vi "Copy Set Default Value - Multiple Converter.vi"(11 "error in":errorcluster) -> (15 "error out":errorcluster)   [LabVIEW 2021, in "Converter.lvlib"]
uses:
  Converter.lvlib
  Path Functions/Path Functions.lvlib
  Converter Reusables/Converter Reusables.lvlib
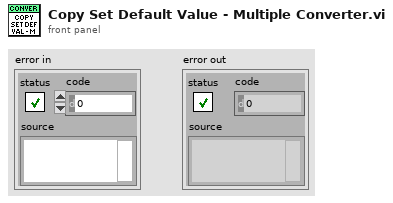
[diagram p1: front panel]
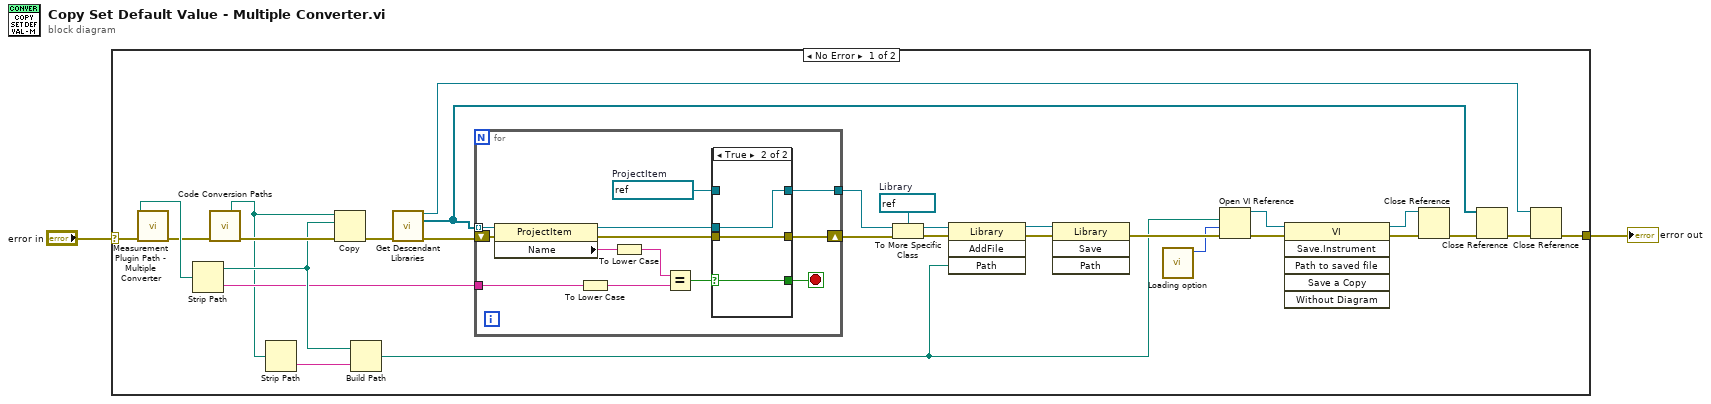
[diagram p0: block diagram]
diagram:
  n1 = case shown="No Error" "error in" {
    selector: "error in" -> [w18 w51]
    tunnel: [w22 w51] -> w2
    frame No Error {
      w12 = refnum<vi> refnum  # Library
      n2 = call "Measurement Plugin Path - Multiple Converter.vi"("error in"=w18) -> ("measurement ui lib"=w19:path, "error out"=w17:errorcluster)  [unwired: 2 in, 11 out]
      n3 = Strip Path(path=w19) -> (stripped path=w29:path, name=w28:string)
      n4 = call "Code Conversion Paths.vi"("error in"=w17) -> ("deafult value setter vi"=w21:path, "error out"=w31:errorcluster)  [unwired: 6 in, 7 out]
      n5 = Strip Path(path=w21) -> (name=w20:string)  [unwired: 1 out]
      n6 = Copy(8:w31, 10:w29, 11:w21) -> (0:w16:errorcluster)  [unwired: 2 in, 2 out]
      n7 = Build Path(base path=w29, name or relative path=w20) -> (appended path=w8:path)
      n8 = call "Get Descendant Libraries.vi"("error in"=w16) -> ("project out"=w23:refnum<vi>, "all descendents"=w27:refnum<vi>[], "error out"=w30:errorcluster)  [unwired: 12 in]
      n9 = for {
        tunnel: w27 -> [w44] mode=indexing
        tunnel: [w37] -> w25
        tunnel: w28 -> [w36]
        shift-right: [w32] -> w10
        shift-left: w30 -> [w35]
        stop <- w38 stop-if-true
        w41 = refnum<vi> refnum  # ProjectItem
        n10 = property class="ProjectItem"(reference=w44, error in=w35) -> (reference out=w40:refnum<vi>, error out=w39:errorcluster, "Name"=w43:string)
        n11 = To Lower Case(string=w36) -> (all lower case string=w33:string)
        n12 = To Lower Case(string=w43) -> (all lower case string=w34:string)
        n13 = Equal?(x=w34, y=w33) -> (x = y?=w42:bool)
        n14 = case shown="True" w42 {
          selector: w42 -> [w46 w49]
          tunnel: w40 -> [_ w50]
          tunnel: [w45 w48] -> w32
          tunnel: [w47 w50] -> w37
          tunnel: w41 -> [w47 _]
          tunnel: [w46 w49] -> w38
          tunnel: w39 -> [w45 w48]
          frame False {
          }
          frame True {
          }
        }
      }
      n15 = To More Specific Class(target class=w12, reference=w25, error in=w10) -> (specific class reference=w11:refnum<vi>, error out=w13:errorcluster)
      n16 = invoke class="Library" method="AddFile"(reference=w11, error in=w13, "Path"=w8) -> (reference out=w15:refnum<vi>, error out=w14:errorcluster)  [unwired: 1 in, 2 out]
      n17 = invoke class="Library" method="Save"(reference=w15, error in=w14) -> (error out=w24:errorcluster)  [unwired: 2 in, 3 out]
      n18 = call "Loading option.vi"() -> ("options"=w7:i32)  [unwired: 11 in]
      n19 = Open VI Reference(vi path=w8, options=w7, error in (no error)=w24) -> (vi reference=w5:refnum<vi>, error out=w9:errorcluster)  [unwired: 3 in]
      n20 = invoke class="VI" method="Save.Instrument"(reference=w5, error in=w9) -> (reference out=w3:refnum<vi>, error out=w6:errorcluster)  [unwired: 4 in, 4 out]
      n21 = Close Reference(reference=w3, error in (no error)=w6) -> (error out=w4:errorcluster)
      n22 = Close Reference(reference=w27, error in (no error)=w4) -> (error out=w26:errorcluster)
      n23 = Close Reference(reference=w23, error in (no error)=w26) -> (error out=w22:errorcluster)
    }
    frame Error {
    }
  }
  "error out" <- w2
